vi "VIH ProjFile - Group Rule - Read.vi"(6 "MasterRule (F)":bool, 8 "error in":errorcluster, 10 "Project Folder":path, 11 "XML Parent Item":refnum<k20>) -> (0 "error out":errorcluster, 1 "Group Rule out":T1, 2 "changed":bool, 3 "dup XML Parent Item":refnum<k20>)   [LabVIEW 2014]
doc: "::: VI Helpeks :::\nCopyright (c) 2000-2026 Konstantin Shifershteyn. All rights reserved."
uses:
  _VIH HelpGen.llb/VIH HelpGen Typedef - Cluster - Group Rule.ctl
  _VIH HelpGen.llb/VIH HelpGen Typedef - Enum - Default,Enable,Disable.ctl
  _VIH HelpGen.llb/VIH HelpGen Typedef - Cluster - Group Rule - Source Paths.ctl
  _VIH HelpGen.llb/VIH HelpGen Typedef - Cluster - Group Rule - Target Paths.ctl
  _VIH HelpGen.llb/VIH HelpGen Typedef - Enum - Description Mode.ctl
  _VIH HelpGen.llb/VIH HelpGen Typedef - Cluster - Control Rule.ctl
  _VIH HelpGen.llb/VIH HelpGen Typedef - Cluster - Enum Value Info.ctl
  _VIH HelpGen.llb/VIH HelpGen Typedef - Cluster - Group Rule - Flags.ctl
  <vilib>/xml/Close Reference(Node).vi
  <vilib>/xml/NI_XML.lvlib
panel:
  in  "Group Rule (data)":T1
  # "VI Helpeks\nCopyright (c) 2012-2026 Konstantin Shifershteyn"
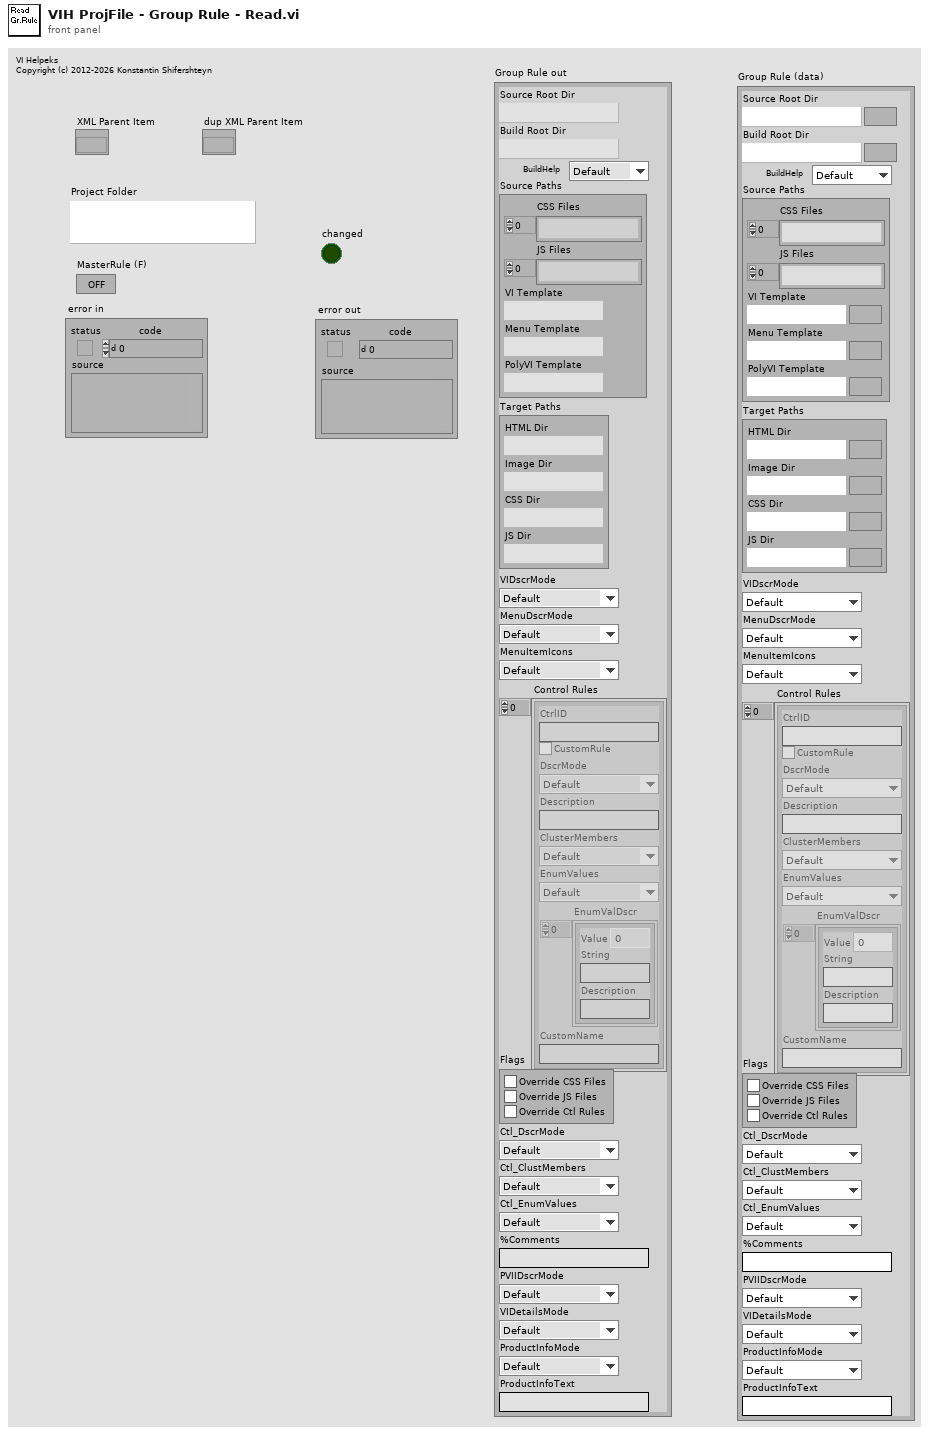
[diagram p1: front panel]
types:
  T1 = typedef "VIH HelpGen Typedef - Cluster - Group Rule.ctl" = cluster{"Source Root Dir":path, "Build Root Dir":path, "BuildHelp":T2, "Source Paths":T3, "Target Paths":T4, "VIDscrMode":T5, "MenuDscrMode":T5, "MenuItemIcons":T2, "Control Rules":T6[], "Flags":T8, "Ctl_DscrMode":T5, "Ctl_ClustMembers":T2, "Ctl_EnumValues":T2, "%Comments":string, "PVIIDscrMode":T5, "VIDetailsMode":T5, "ProductInfoMode":T2, "ProductInfoText":string}
  T2 = typedef "VIH HelpGen Typedef - Enum - Default,Enable,Disable.ctl" = enum16{"Default", "Enable", "Disable"}
  T3 = typedef "VIH HelpGen Typedef - Cluster - Group Rule - Source Paths.ctl" = cluster{"CSS Files":path[], "JS Files":path[], "VI Template":path, "Menu Template":path, "PolyVI Template":path}
  T4 = typedef "VIH HelpGen Typedef - Cluster - Group Rule - Target Paths.ctl" = cluster{"HTML Dir":path, "Image Dir":path, "CSS Dir":path, "JS Dir":path}
  T5 = typedef "VIH HelpGen Typedef - Enum - Description Mode.ctl" = enum16{"Default", "Description", "Description1", "Description2", "Custom", "None"}
  T6 = typedef "VIH HelpGen Typedef - Cluster - Control Rule.ctl" = cluster{"CtrlID":string, "CustomRule":bool, "DscrMode":T5, "Description":string, "ClusterMembers":T2, "EnumValues":T2, "EnumValDscr":T7[], "CustomName":string}
  T7 = typedef "VIH HelpGen Typedef - Cluster - Enum Value Info.ctl" = cluster{"Value":ext, "String":string, "Description":string}
  T8 = typedef "VIH HelpGen Typedef - Cluster - Group Rule - Flags.ctl" = cluster{"Override CSS Files":bool, "Override JS Files":bool, "Override Ctl Rules":bool}
  T9 = typedef "KS HelpGen Typedef - Cluster - Group Rule.ctl" = cluster{"Source Root Dir":path, "Build Root Dir":path, "BuildHelp":T10, "Source Paths":T11, "Target Paths":T12, "VIDscrMode":T13, "MenuDscrMode":T13, "MenuItemIcons":T10, "Control Rules":T14[], "Flags":T16, "Ctl_DscrMode":T13, "Ctl_ClustMembers":T10, "Ctl_EnumValues":T10, "%Comments":string, "PVIIDscrMode":T13, "VIDetailsMode":T13, "ProductInfoMode":T10, "ProductInfoText":string}
  T10 = typedef "KS HelpGen Typedef - Enum - Default,Enable,Disable.ctl" = enum16{"Default", "Enable", "Disable"}
  T11 = typedef "KS HelpGen Typedef - Cluster - Group Rule - Source Paths.ctl" = cluster{"CSS Files":path[], "JS Files":path[], "VI Template":path, "Menu Template":path, "PolyVI Template":path}
  T12 = typedef "KS HelpGen Typedef - Cluster - Group Rule - Target Paths.ctl" = cluster{"HTML Dir":path, "Image Dir":path, "CSS Dir":path, "JS Dir":path}
  T13 = typedef "KS HelpGen Typedef - Enum - Description Mode.ctl" = enum16{"Default", "Description", "Description1", "Description2", "Custom", "None"}
  T14 = typedef "KS HelpGen Typedef - Cluster - Control Rule.ctl" = cluster{"CtrlID":string, "CustomRule":bool, "DscrMode":T13, "Description":string, "ClusterMembers":T10, "EnumValues":T10, "EnumValDscr":T15[], "CustomName":string}
  T15 = typedef "KS HelpGen Typedef - Cluster - Enum Value Info.ctl" = cluster{"Value":ext, "String":string, "Description":string}
  T16 = typedef "KS HelpGen Typedef - Cluster - Group Rule - Flags.ctl" = cluster{"Override CSS Files":bool, "Override JS Files":bool, "Override Ctl Rules":bool}
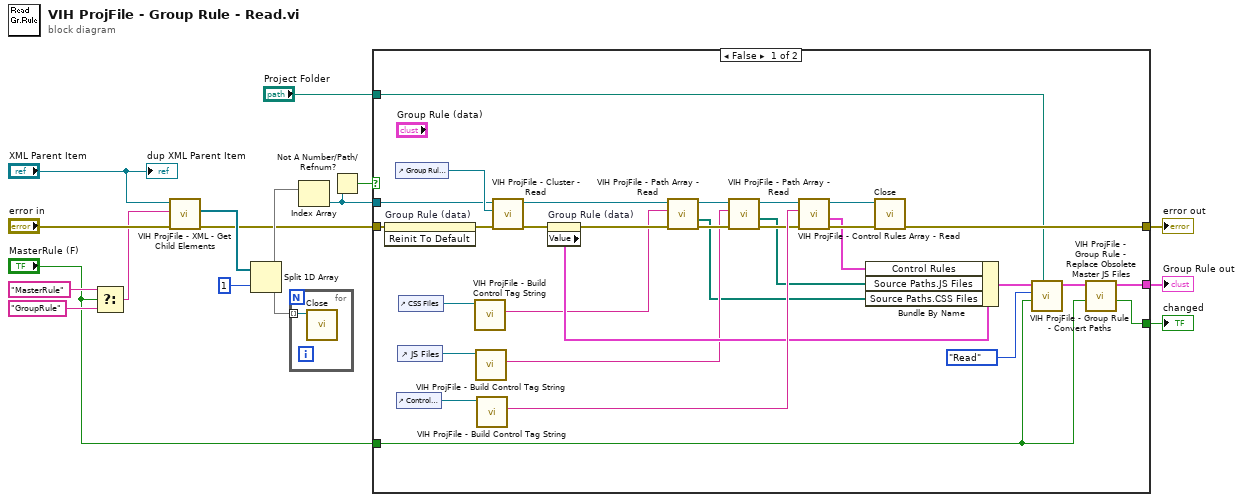
[diagram p0: block diagram]
diagram:
  n1 = Select(t="MasterRule" ("Tag Name"), s="MasterRule (F)", f="GroupRule") -> (s? t:f=w3:string)
  n2 = call "VIH ProjFile - XML - Get Child Elements.vi"("error in"="error in", "Tag Name"=w3, "XML Parent Item"="XML Parent Item") -> ("error out"=w5:errorcluster, "Array of Elements"=w6:refnum<k20>[])  [unwired: 6 in, 1 out]
  n3 = Split 1D Array(array=w6, index=1) -> (first subarray=w12:refnum<k20>[], second subarray=w11:refnum<k20>[])
  n4 = for {
    tunnel: w11 -> [w18] mode=indexing
    n5 = call-poly <vilib>:"Close.vi"("node"=w18) -> ()  [unwired: 8 in, 1 out]
  }
  n6 = Index Array(array=w12) -> (element=w15:refnum<k20>)  [unwired: 1 in]
  n7 = Not A Number/Path/Refnum?(number/path/refnum=w15) -> (NaN/Path/Refnum?=w14:bool)
  n8 = case shown="False" w14 {
    tunnel: w5 -> [w47 w50]
    tunnel: [w43 w50] -> w17
    tunnel: [w21 _] -> w16
    tunnel: w15 -> [w29 _]
    tunnel: "Project Folder" -> [w25 _]
    tunnel: "MasterRule (F)" -> [w20 _]
    tunnel: [w19 _] -> w1
    frame False {
      n9 = invoke on="Group Rule (data)" class="Clust (strict)" method="Reinit To Default"(error in=w47) -> (error out=w48:errorcluster)  [unwired: 2 in, 2 out]
      n10 = control-ref of="Group Rule (data)"() -> (w49:refnum<vi>)
      n11 = control-ref of="Control Rules"() -> (w26:refnum<vi>)
      n12 = control-ref of="JS Files"() -> (w27:refnum<vi>)
      n13 = control-ref of="CSS Files"() -> (w28:refnum<vi>)
      n14 = call "VIH ProjFile - Build Control Tag String.vi"("Ctl Refnum"=w28) -> ("Control Tag"=w33:string)  [unwired: 6 in, 4 out]
      n15 = call "VIH ProjFile - Build Control Tag String.vi"("Ctl Refnum"=w27) -> ("Control Tag"=w32:string)  [unwired: 6 in, 4 out]
      n16 = call "VIH ProjFile - Build Control Tag String.vi"("Ctl Refnum"=w26) -> ("Control Tag"=w44:string)  [unwired: 6 in, 4 out]
      n17 = call "VIH ProjFile - Cluster - Read.vi"("error in"=w48, "Ctl Refnum"=w49, "XML Parent Item"=w29) -> ("error out"=w42:errorcluster, "dup XML Parent Item"=w39:refnum<k20>)  [unwired: 7 in]
      n18 = property on="Group Rule (data)" class="Clust (strict)"(error in=w42) -> (error out=w36:errorcluster, "Value"=w41:T9)  [unwired: 1 in, 1 out]
      n19 = call "VIH ProjFile - Path Array - Read.vi"("error in"=w36, "Property Name"=w33, "XML Parent Item"=w39) -> ("error out"=w35:errorcluster, "Files"=w30:path[], "dup XML Parent Item"=w38:refnum<k20>)  [unwired: 6 in]
      n20 = call "VIH ProjFile - Path Array - Read.vi"("error in"=w35, "Property Name"=w32, "XML Parent Item"=w38) -> ("error out"=w34:errorcluster, "Files"=w31:path[], "dup XML Parent Item"=w37:refnum<k20>)  [unwired: 6 in]
      n21 = call "VIH ProjFile - Control Rules Array - Read.vi"("error in"=w34, "Property Name"=w44, "XML Parent Item"=w37) -> ("error out"=w45:errorcluster, "Control Rules"=w40:T6[], "dup XML Parent Item"=w46:refnum<k20>)  [unwired: 5 in, 1 out]
      n22 = Bundle By Name(cluster=w41, "Control Rules"=w40, "Source Paths.JS Files"=w31, "Source Paths.CSS Files"=w30) -> (w24:T9)
      n23 = call-poly <vilib>:"Close.vi"("error in (no error)"=w45, "node"=w46) -> ("error out"=w43:errorcluster)  [unwired: 7 in]
      n24 = call "VIH ProjFile - Group Rule - Convert Paths.vi"("Root Dir"=w25, "Master Rule (F)"=w20, "Operation"=enum16{"Read", "Write"}."Read", "Group Rule"=w24) -> ("Group Rule out"=w22:T1)  [unwired: 7 in]
      n25 = call "VIH ProjFile - Group Rule - Replace Obsolete Master JS Files.vi"("Master Rule (F)"=w20, "Group Rule"=w22) -> ("changed"=w19:bool, "Group Rule out"=w21:T1)  [unwired: 8 in]
    }
    frame True {
    }
  }
  "error out" <- w17
  "Group Rule out" <- w16
  "changed" <- w1
  "dup XML Parent Item" <- "XML Parent Item"
